vi "Main.vi"() -> ()   [LabVIEW 2026]
uses:
  <vilib>/Instr/_visa.llb/VISA Configure Serial Port (Instr).vi
panel:
  in  "EMERGENCIA":bool
  in  "PWM":dbl min=0.0 max=100.0
  out "SP Vs ALTURA":cluster{dbl, dbl}(graph)
  out "PING PONG":dbl(slide) scale=0.0..50.0
  out "PID":enum16{"NO CONFIGURADO", "CONFIGURADO"}(ring)
  out "error out":errorcluster
  out "Enum":enum16{"DESCONECTADO", "CONECTADO"}(ring)
  out "ESTADO  SYS":enum16{"DETENIDO", "EJECUTANDO", "ERROR"}(ring)
  out "MAQUINA DE ESTADOS":T1(ring)
  in  "PARADA":bool
  in  "INICIO":bool
  out "PID":string
  in  "SP":dbl min=0.0 max=100.0
  in  "KD":dbl=0.07 min=0.0 max=65535.0
  in  "KI":dbl=0.14 min=0.0 max=65535.0
  in  "KP":dbl=3.9 min=0.0 max=65535.0
  in  "Parametros":bool
  out "SALIDA PID":dbl format="%.2g"
  out "ERROR":dbl format="%.2g"
  out "ALTURA":dbl format="%.2g"
  out "SP":dbl format="%.2f"
  out "array":string[][](array[string])
  out "Procesar":string
  in  "Stop Simulation":bool
  in  "Numeric":u32=115200
  in  "VISA resource name":refnum<visa-resource-name>="COM12"
  out "Iteracion":i32
  # "Sistema Levitador Neumático"
  # "Planta"
  # "Grafico en Tiempo Real"
  # "COMUNICACIÓN"
  # "ESTADO DEL SISTEMA"
  # "Estado :"
  # "Puerto :"
  # "Comunicación :"
  # "Baud :"
  # "Estado PID :"
  # "CONFIGURACIÓN PID"
  # "VARIABLES EN TIEMPO REAL"
  # "KP :"
  # "KI  :"
  # "KD :"
  # "SP :"
  # "Mensaje a Procesar :"
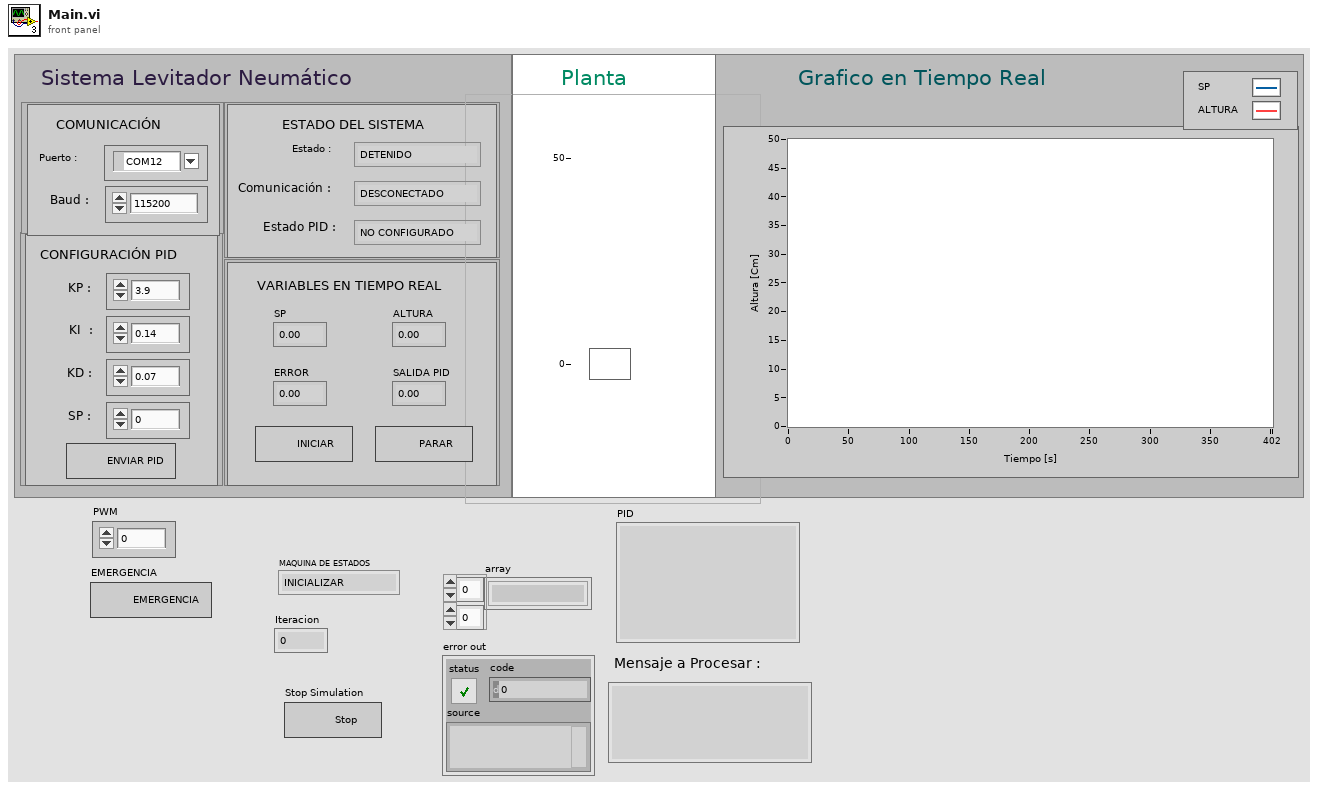
[diagram p1: front panel]
types:
  T1 = enum16{"INICIALIZAR", "ESPERA", "RECIBIR", "PROCESAR", "ENVIAR_RUN", "ENVIAR_STOP", "ENVIAR_PID", "ERROR", "CERRAR"}
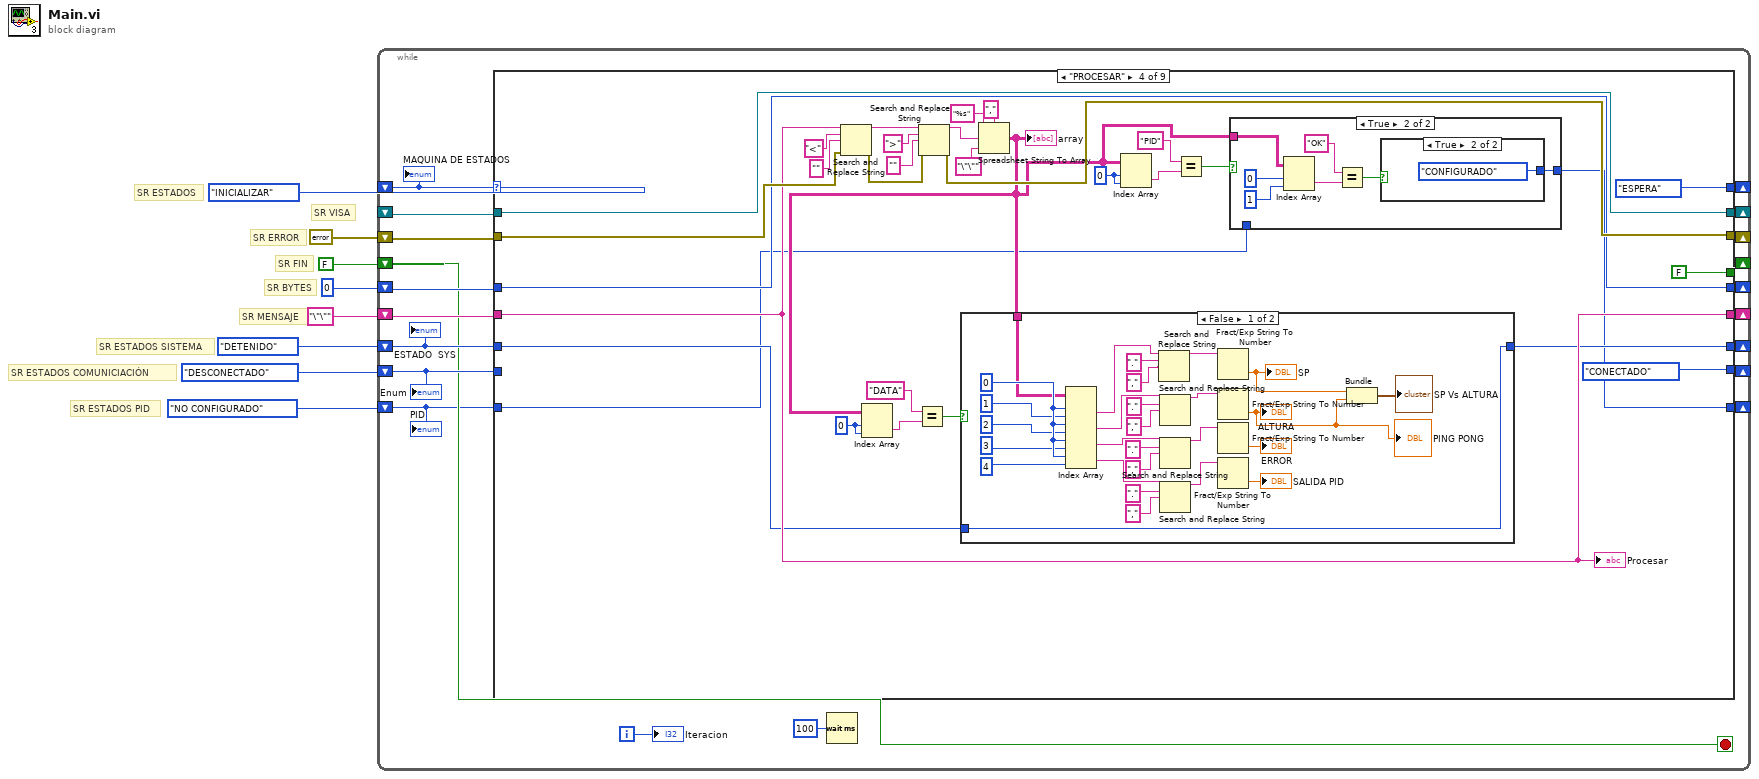
[diagram p0: block diagram]
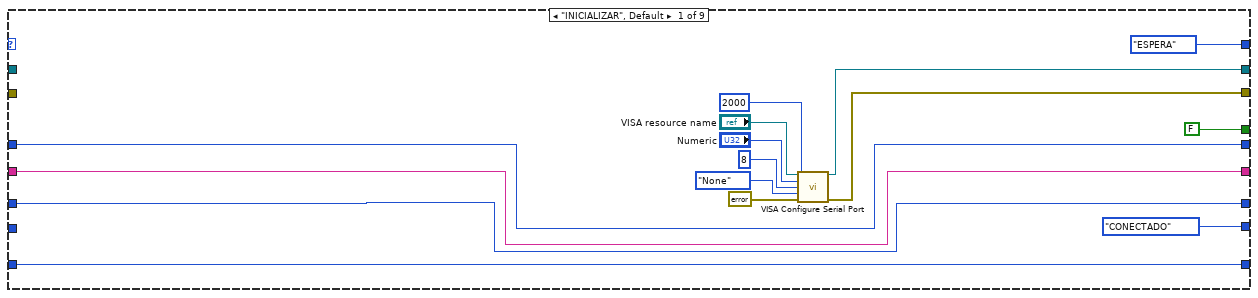
[diagram p2: hidden frame]
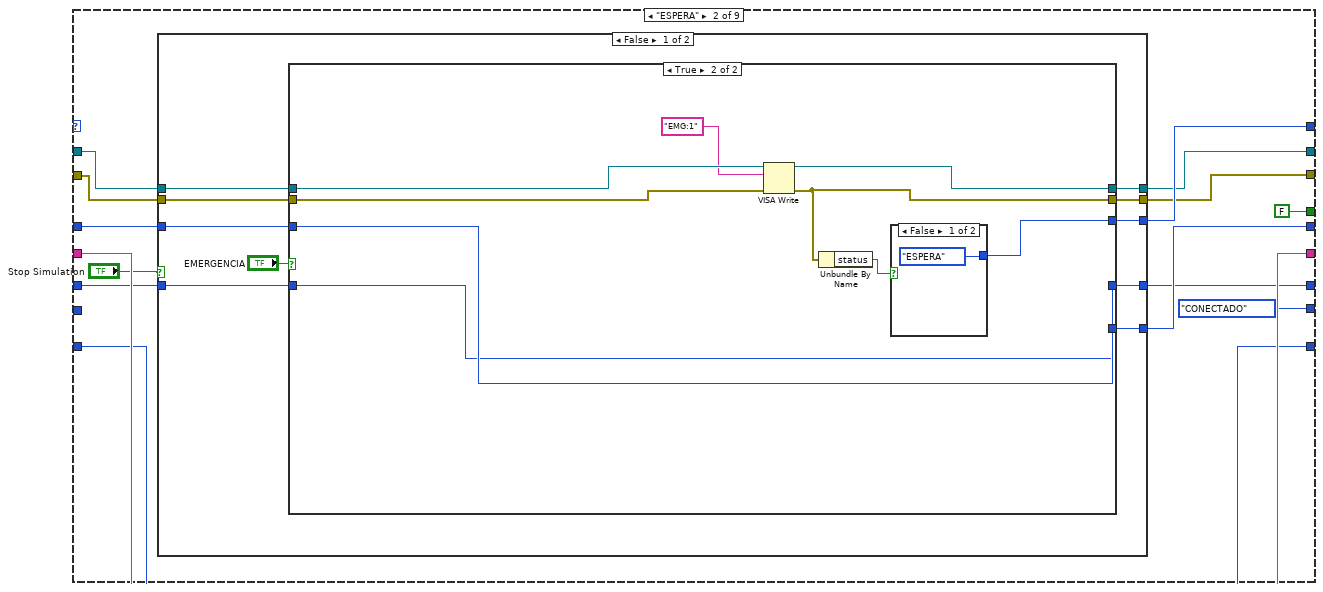
[diagram p3: hidden frame]
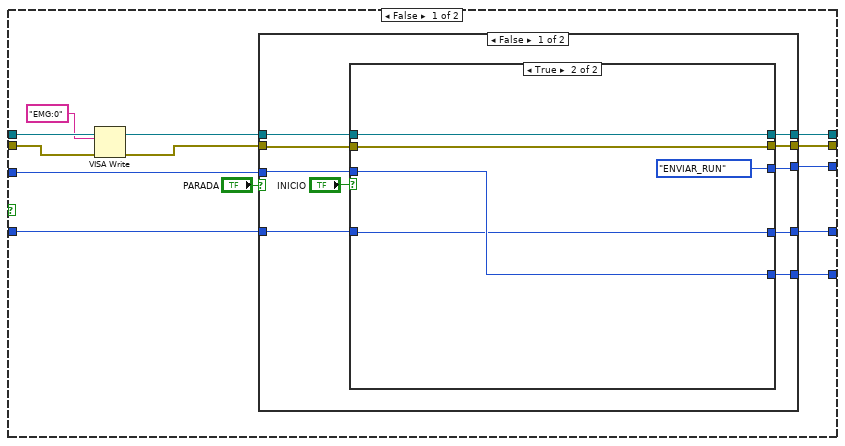
[diagram p4: hidden frame]
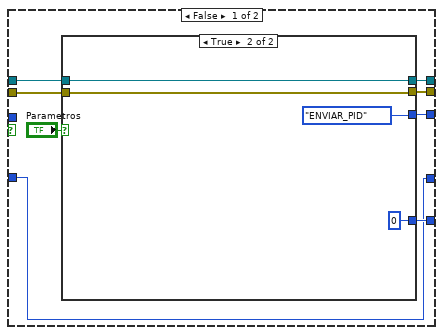
[diagram p5: hidden frame]
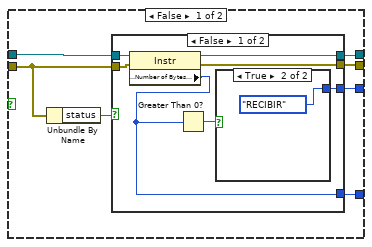
[diagram p6: hidden frame]
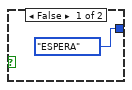
[diagram p7: hidden frame]
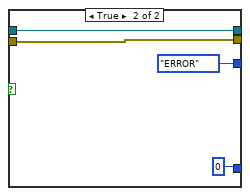
[diagram p8: hidden frame]
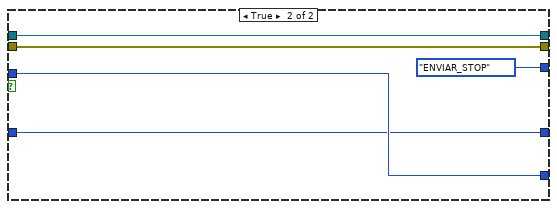
[diagram p9: hidden frame]
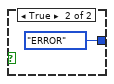
[diagram p10: hidden frame]
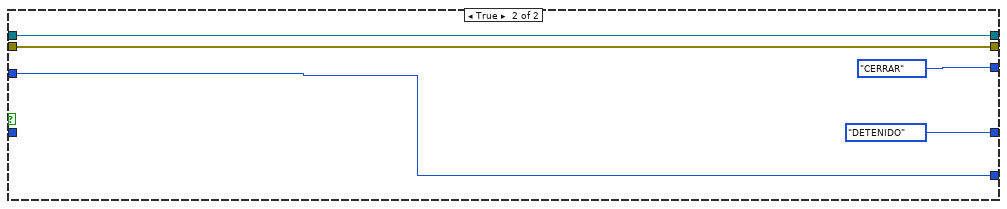
[diagram p11: hidden frame]
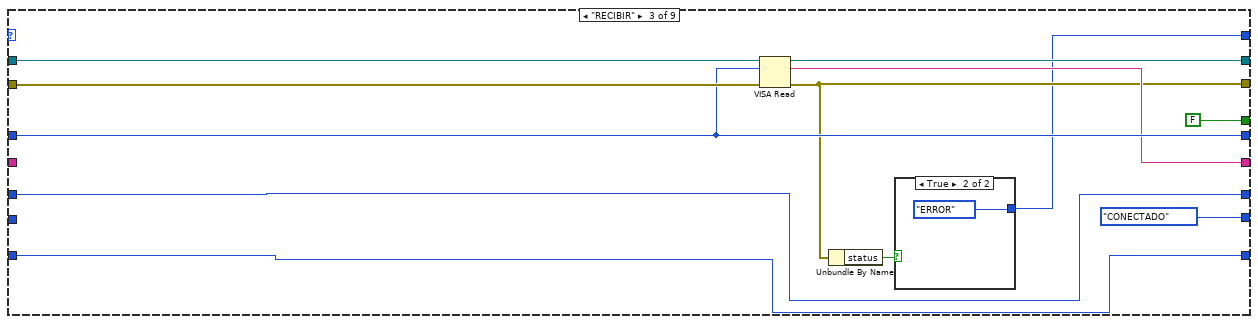
[diagram p12: hidden frame]
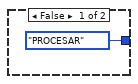
[diagram p13: hidden frame]
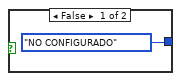
[diagram p15: hidden frame]
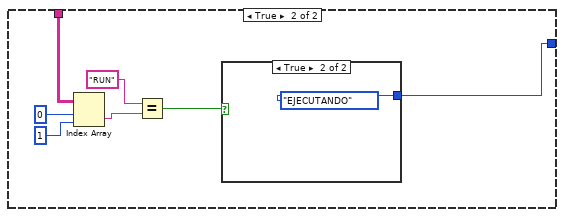
[diagram p16: hidden frame]
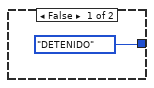
[diagram p17: hidden frame]
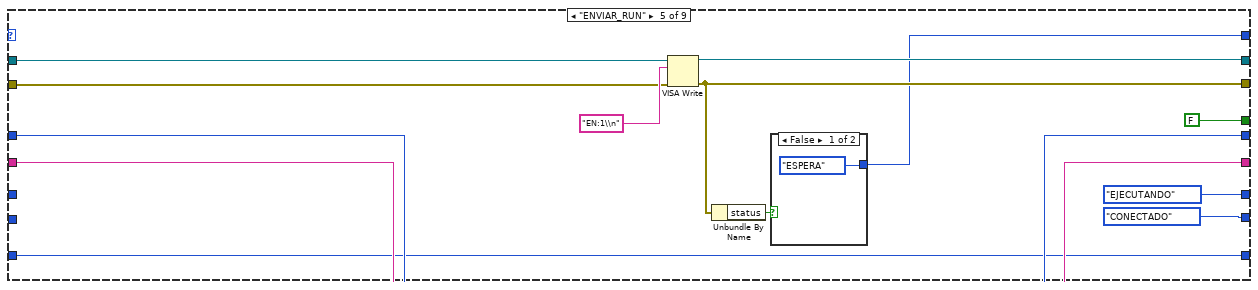
[diagram p18: hidden frame]
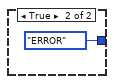
[diagram p19: hidden frame]
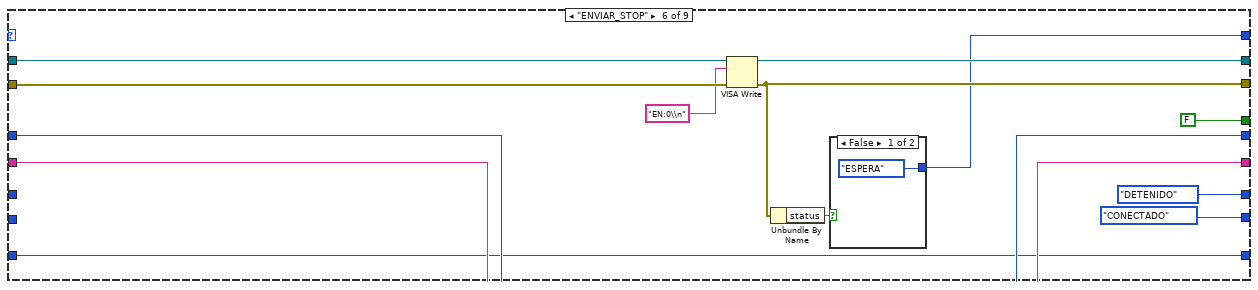
[diagram p20: hidden frame]
diagram:
  # "SR ESTADOS PID"
  # "SR ESTADOS COMUNICIACIÓN"
  # "SR ESTADOS SISTEMA"
  # "SR MENSAJE"
  # "SR BYTES"
  # "SR FIN"
  # "SR ERROR"
  # "SR ESTADOS"
  # "SR VISA"
  n1 = while {
    shift-right: [w16] -> _
    shift-left: T1."INICIALIZAR" -> [w17]
    shift-right: [w26] -> _
    shift-left: _ -> [w24]
    shift-right: [w25] -> _
    shift-left: errorcluster {"status"=FALSE, "code"=0, "source"=""} ("error out") -> [w23]
    shift-right: [w22] -> _
    shift-left: FALSE -> [w11]
    shift-right: [w21] -> _
    shift-left: u32 0 ("Bytes at Port") -> [w20]
    shift-right: [w19] -> _
    shift-left: "\"\"" -> [w18]
    shift-right: [w12] -> _
    shift-left: enum16{"DETENIDO", "EJECUTANDO", "ERROR"}."DETENIDO" -> [w14]
    shift-right: [w13] -> _
    shift-left: enum16{"DESCONECTADO", "CONECTADO"}."DESCONECTADO" -> [w15]
    shift-right: [w9] -> _
    shift-left: enum16{"NO CONFIGURADO", "CONFIGURADO"}."NO CONFIGURADO" -> [w10]
    i -> [w28]
    stop <- w11 stop-if-true
    n2 = case shown="\"PROCESAR\"" w17 {
      tunnel: [T1."ESPERA" w57 w152 T1."ESPERA" w247 w260 w289 T1."CERRAR" T1."CERRAR"] -> w16
      tunnel: [w37 w54 w157 w193 w249 w261 w294 w311 w313] -> w26
      tunnel: [w36 w53 w154 w184 w248 w262 w291 w305 w314] -> w25
      tunnel: w24 -> [_ w55 w159 w193 w251 w266 w295 w311 w313]
      tunnel: w23 -> [_ w49 w158 w185 w250 w265 w297 w305 w315]
      tunnel: [FALSE FALSE FALSE FALSE FALSE FALSE FALSE FALSE TRUE] -> w22
      tunnel: [w34 w52 w156 w180 w244 w263 w299 w309 w320] -> w21
      tunnel: w20 -> [w34 w51 w156 w180 w244 w263 w299 w309 w320]
      tunnel: [w33 w50 w155 w176 w245 w264 w298 w308 w319] -> w19
      tunnel: w18 -> [w33 w50 _ w176 w245 w264 w298 w308 w319]
      tunnel: w14 -> [w30 w46 w150 w170 _ _ w287 w304 _]
      tunnel: w15 -> [_ _ _ _ _ _ _ _ _]
      tunnel: [enum16{"DESCONECTADO", "CONECTADO"}."CONECTADO" enum16{"DESCONECTADO", "CONECTADO"}."CONECTADO" enum16{"DESCONECTADO", "CONECTADO"}."CONECTADO" enum16{"DESCONECTADO", "CONECTADO"}."CONECTADO" enum16{"DESCONECTADO", "CONECTADO"}."CONECTADO" enum16{"DESCONECTADO", "CONECTADO"}."CONECTADO" enum16{"DESCONECTADO", "CONECTADO"}."CONECTADO" enum16{"DESCONECTADO", "CONECTADO"}."CONECTADO" enum16{"DESCONECTADO", "CONECTADO"}."DESCONECTADO"] -> w13
      tunnel: [w30 w47 w150 w171 enum16{"DETENIDO", "EJECUTANDO", "ERROR"}."EJECUTANDO" enum16{"DETENIDO", "EJECUTANDO", "ERROR"}."DETENIDO" w287 w304 enum16{"DETENIDO", "EJECUTANDO", "ERROR"}."DETENIDO"] -> w12
      tunnel: w10 -> [w29 w44 w149 w163 w241 w256 w286 w303 w312]
      tunnel: [w29 w44 w149 w164 w241 w256 w286 w303 w312] -> w9
      frame "INICIALIZAR", Default {
        n3 = call-poly "VISA Configure Serial Port"("VISA resource name"="VISA resource name", "timeout (10sec)"=u32 2000, "baud rate (9600)"="Numeric", "data bits (8)"=u16 8, "parity (0:none)"=enum16{"None", "Odd", "Even", "Mark", "Space"}."None", "error in (no error)"=errorcluster {"status"=FALSE, "code"=0, "source"=""}) -> ("VISA resource name out"=w37:refnum<visa-resource-name>, "error out"=w36:errorcluster)  [unwired: 8 in]
      }
      frame "ESPERA" {
        n4 = case shown="False" "Stop Simulation" {
          tunnel: [w67 T1."CERRAR"] -> w57
          tunnel: w55 -> [w66 w145]
          tunnel: [w65 w145] -> w54
          tunnel: [w64 w144] -> w53
          tunnel: [w63 w147] -> w52
          tunnel: w51 -> [w62 w147]
          tunnel: w49 -> [w61 w144]
          tunnel: [w60 enum16{"DETENIDO", "EJECUTANDO", "ERROR"}."DETENIDO"] -> w47
          tunnel: w46 -> [w59 _]
          frame False {
            n5 = case shown="True" "EMERGENCIA" {
              tunnel: [w80 w136] -> w67
              tunnel: w66 -> [w72 w138]
              tunnel: [w79 w133] -> w65
              tunnel: [w78 w134] -> w64
              tunnel: [w77 w141] -> w63
              tunnel: w62 -> [w76 w141]
              tunnel: w61 -> [w71 w137]
              tunnel: [w74 w140] -> w60
              tunnel: w59 -> [w73 w140]
              frame False {
                n6 = VISA Write(VISA resource name=w72, write buffer="EMG:0", error in (no error)=w71) -> (VISA resource name out=w69:refnum<visa-resource-name>, error out=w68:errorcluster)  [unwired: 1 out]
                n7 = case shown="False" "PARADA" {
                  tunnel: [w90 T1."ENVIAR_STOP"] -> w80
                  tunnel: w69 -> [w89 w132]
                  tunnel: w68 -> [w88 w131]
                  tunnel: [w87 w132] -> w79
                  tunnel: [w86 w131] -> w78
                  tunnel: [w85 w130] -> w77
                  tunnel: w76 -> [w83 w130]
                  tunnel: [w82 w128] -> w74
                  tunnel: w73 -> [w81 w128]
                  frame False {
                    n8 = case shown="True" "INICIO" {
                      tunnel: [w98 T1."ENVIAR_RUN"] -> w90
                      tunnel: w89 -> [w96 w126]
                      tunnel: w88 -> [w95 w125]
                      tunnel: [w94 w126] -> w87
                      tunnel: [w93 w125] -> w86
                      tunnel: [w92 w124] -> w85
                      tunnel: w83 -> [_ w124]
                      tunnel: [w91 w123] -> w82
                      tunnel: w81 -> [w91 w123]
                      frame False {
                        n9 = case shown="True" "Parametros" {
                          tunnel: [w105 T1."ENVIAR_PID"] -> w98
                          tunnel: w96 -> [w104 w121]
                          tunnel: w95 -> [w100 w120]
                          tunnel: [w103 w121] -> w94
                          tunnel: [w102 w120] -> w93
                          tunnel: [w101 u32 0 ("Bytes at Port")] -> w92
                          frame False {
                            n10 = Unbundle By Name(w100) -> ("status"=w99:bool)
                            n11 = case shown="False" w99 {
                              tunnel: [w112 T1."ERROR"] -> w105
                              tunnel: w104 -> [w111 w118]
                              tunnel: w100 -> [w110 w117]
                              tunnel: [w109 w118] -> w103
                              tunnel: [w108 w117] -> w102
                              tunnel: [w106 u32 0 ("Bytes at Port")] -> w101
                              frame False {
                                n12 = property class="Instr"(reference=w111, error in=w110) -> (reference out=w109:refnum<visa-resource-name>, error out=w108:errorcluster, "Serial Settings:Number of Bytes at Serial Port"=w106:u32)
                                n13 = Greater Than 0?(x=w106) -> (x > 0?=w107:bool)
                                n14 = case shown="True" w107 {
                                tunnel: [T1."ESPERA" T1."RECIBIR"] -> w112
                                frame False {
                                }
                                frame True {
                                }
                                }
                              }
                              frame True {
                              }
                            }
                          }
                          frame True {
                          }
                        }
                      }
                      frame True {
                      }
                    }
                  }
                  frame True {
                  }
                }
              }
              frame True {
                n15 = VISA Write(VISA resource name=w138, write buffer="EMG:1", error in (no error)=w137) -> (VISA resource name out=w133:refnum<visa-resource-name>, error out=w134:errorcluster)  [unwired: 1 out]
                n16 = Unbundle By Name(w134) -> ("status"=w139:bool)
                n17 = case shown="False" w139 {
                  tunnel: [T1."ESPERA" T1."ERROR"] -> w136
                  frame False {
                  }
                  frame True {
                  }
                }
              }
            }
          }
          frame True {
          }
        }
      }
      frame "RECIBIR" {
        n18 = VISA Read(VISA resource name=w159, byte count=w156, error in (no error)=w158) -> (VISA resource name out=w157:refnum<visa-resource-name>, read buffer=w155:string, error out=w154:errorcluster)  [unwired: 1 out]
        n19 = Unbundle By Name(w154) -> ("status"=w153:bool)
        n20 = case shown="True" w153 {
          tunnel: [T1."PROCESAR" T1."ERROR"] -> w152
          frame False {
          }
          frame True {
          }
        }
      }
      frame "PROCESAR" {
        w169 = 0 ("index (row)")
        w175 = 0 ("index (row)")
        n21 = Search and Replace String(input string=w176, search string="<", replace string="" ("replace string (\"\")"), error in=w185) -> (result string=w189:string, error out=w188:errorcluster)  [unwired: 4 in, 2 out]
        n22 = Search and Replace String(input string=w189, search string=">", replace string="" ("replace string (\"\")"), error in=w188) -> (result string=w182:string, error out=w184:errorcluster)  [unwired: 4 in, 2 out]
        n23 = Spreadsheet String To Array(delimiter (Tab)=",", format string="%s", spreadsheet string=w182, array type (2D Dbl)="\"\"") -> (array=w165:string[][])
        "array" <- w165
        n24 = Index Array(array=w165, index (row)=w175, index (col)=w175) -> (element=w174:string)
        n25 = Equal?(x="DATA", y=w174) -> (x = y?=w172:bool)
        n26 = case shown="False" w172 {
          tunnel: w165 -> [w206 w238]
          tunnel: [w205 w232] -> w171
          tunnel: w170 -> [w205 _]
          frame False {
            w231 = 0 ("index (row)")
            n27 = Index Array(array=w206, index (row) #1=w231, index (col) #1=1 ("index"), index (row) #2=w231, index (col) #2=2 ("index"), index (row) #3=w231, index (col) #3=3 ("index"), index (row) #4=w231, index (col) #4=4 ("index")) -> (element #1=w225:string, element #2=w216:string, element #3=w215:string, element #4=w214:string)
            n28 = Search and Replace String(input string=w225, search string=".", replace string="," ("replace string (\"\")")) -> (result string=w223:string)  [unwired: 5 in, 3 out]
            n29 = Search and Replace String(input string=w216, search string=".", replace string="," ("replace string (\"\")")) -> (result string=w212:string)  [unwired: 5 in, 3 out]
            n30 = Search and Replace String(input string=w215, search string=".", replace string="," ("replace string (\"\")")) -> (result string=w211:string)  [unwired: 5 in, 3 out]
            n31 = Search and Replace String(input string=w214, search string=".", replace string="," ("replace string (\"\")")) -> (result string=w210:string)  [unwired: 5 in, 3 out]
            n32 = Fract/Exp String To Number(string=w223) -> (number=w208:dbl)  [unwired: 3 in, 1 out]
            "SP" <- w208
            n33 = Fract/Exp String To Number(string=w212) -> (number=w204:dbl)  [unwired: 3 in, 1 out]
            "ALTURA" <- w204
            "PING PONG" <- w204
            n34 = Fract/Exp String To Number(string=w211) -> (number=→"ERROR":dbl)  [unwired: 3 in, 1 out]
            n35 = Fract/Exp String To Number(string=w210) -> (number=→"SALIDA PID":dbl)  [unwired: 3 in, 1 out]
            n36 = Bundle(w208, w204) -> (→"SP Vs ALTURA":cluster{dbl, dbl})  [unwired: 1 in]
          }
          frame True {
            n37 = Index Array(array=w238, index (row)=0, index (col)=1 ("disabled index (col)")) -> (element=w235:string)
            n38 = Equal?(x="RUN", y=w235) -> (x = y?=w233:bool)
            n39 = case shown="True" w233 {
              tunnel: [enum16{"DETENIDO", "EJECUTANDO", "ERROR"}."DETENIDO" enum16{"DETENIDO", "EJECUTANDO", "ERROR"}."EJECUTANDO"] -> w232
              frame False {
              }
              frame True {
              }
            }
          }
        }
        n40 = Index Array(array=w165, index (row)=w169, index (col)=w169) -> (element=w168:string)
        n41 = Equal?(x="PID", y=w168) -> (x = y?=w166:bool)
        n42 = case shown="True" w166 {
          tunnel: w165 -> [_ w197]
          tunnel: [w194 w195] -> w164
          tunnel: w163 -> [w194 _]
          frame False {
          }
          frame True {
            n43 = Index Array(array=w197, index (row)=0, index (col)=1 ("disabled index (col)")) -> (element=w199:string)
            n44 = Equal?(x="OK", y=w199) -> (x = y?=w196:bool)
            n45 = case shown="True" w196 {
              tunnel: [enum16{"NO CONFIGURADO", "CONFIGURADO"}."NO CONFIGURADO" enum16{"NO CONFIGURADO", "CONFIGURADO"}."CONFIGURADO"] -> w195
              frame False {
              }
              frame True {
              }
            }
          }
        }
        "Procesar" <- w176
      }
      frame "ENVIAR_RUN" {
        n46 = VISA Write(VISA resource name=w251, write buffer="EN:1\\n", error in (no error)=w250) -> (VISA resource name out=w249:refnum<visa-resource-name>, error out=w248:errorcluster)  [unwired: 1 out]
        n47 = Unbundle By Name(w248) -> ("status"=w253:bool)
        n48 = case shown="False" w253 {
          tunnel: [T1."ESPERA" T1."ERROR"] -> w247
          frame False {
          }
          frame True {
          }
        }
      }
      frame "ENVIAR_STOP" {
        n49 = VISA Write(VISA resource name=w266, write buffer="EN:0\\n", error in (no error)=w265) -> (VISA resource name out=w261:refnum<visa-resource-name>, error out=w262:errorcluster)  [unwired: 1 out]
        n50 = Unbundle By Name(w262) -> ("status"=w268:bool)
        n51 = case shown="False" w268 {
          tunnel: [T1."ESPERA" T1."ERROR"] -> w260
          frame False {
          }
          frame True {
          }
        }
      }
      frame "ENVIAR_PID" {
        n52 = Multiply(x=10.0, y="SP") -> (x*y=w274:dbl)
        n53 = Multiply(x=100.0, y="KP") -> (x*y=w277:dbl)
        n54 = Multiply(x=100.0, y="KI") -> (x*y=w281:dbl)
        n55 = Multiply(x=100.0, y="KD") -> (x*y=w285:dbl)
        n56 = Multiply(x=10.0, y="PWM") -> (x*y=w271:dbl)
        n57 = Format Into String(format string="%.;KP:%d\\nKI:%d\\nKD:%d\\nSP:%d\\nPWM:%d\\n", error in=w297, w277, w281, w285, w274, w271) -> (resulting string=w296:string, error out=w292:errorcluster)  [unwired: 1 in]
        "PID" <- w296
        n58 = VISA Write(VISA resource name=w295, write buffer=w296, error in (no error)=w292) -> (VISA resource name out=w294:refnum<visa-resource-name>, error out=w291:errorcluster)  [unwired: 1 out]
        n59 = Unbundle By Name(w291) -> ("status"=w290:bool)
        n60 = case shown="True" w290 {
          tunnel: [T1."ESPERA" T1."ERROR"] -> w289
          frame False {
          }
          frame True {
          }
        }
      }
      frame "ERROR" {
        "error out" <- w305
      }
      frame "CERRAR" {
        n61 = VISA Close(VISA resource name=w313, error in (no error)=w315) -> (error out=w314:errorcluster)
      }
    }
    n62 = Wait (ms)(milliseconds to wait=u32 100) -> ()  [unwired: 1 out]
    "Iteracion" <- w28
    "MAQUINA DE ESTADOS" <- w17
    "ESTADO  SYS" <- w14
    "Enum" <- w15
    "PID" <- w10
  }
